vi "Device_connection_info.vi"(11 "Array":string[](array[string])=["COM7", "", "", "COM6"]) -> (3 "Array 3":string[](array[string]))   [LabVIEW 2021]
panel:
  in  "Array 2":string[](array[string])=["Main Crl is not connnected", "Rs485_1 is not connecetd", "RS485_2 is not connected", "RS422 is not connected"]
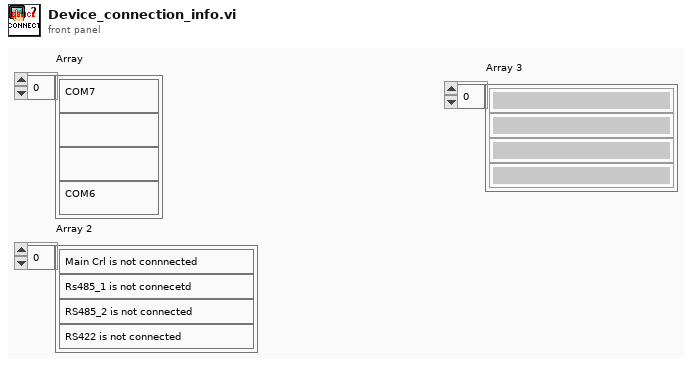
[diagram p1: front panel]
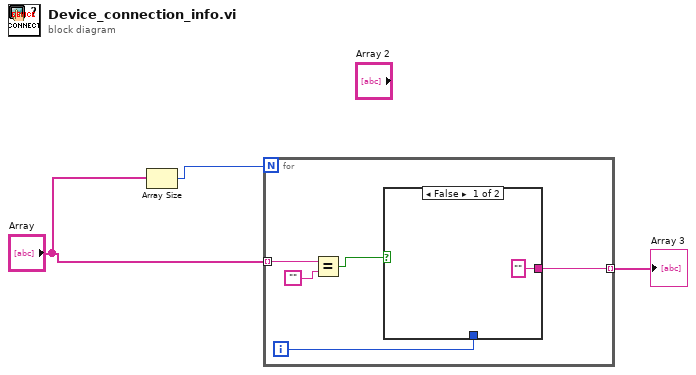
[diagram p0: block diagram]
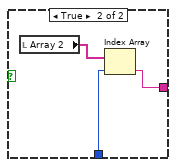
[diagram p2: hidden frame]
diagram:
  n1 = Array Size(array="Array") -> (size(s)=w3:i32)
  n2 = for {
    N: w3 -> [_]
    tunnel: "Array" -> [w8] mode=indexing
    tunnel: [w4] -> w1 mode=indexing
    i -> [w5]
    n3 = Equal?(x=w8, y="") -> (x = y?=w6:bool)
    n4 = case shown="False" w6 {
      tunnel: w5 -> [_ w11]
      tunnel: ["" w10] -> w4
      frame False {
      }
      frame True {
        n5 = local read "Array 2"() -> (w12:string[])
        n6 = Index Array(array=w12, index=w11) -> (element=w10:string)
      }
    }
  }
  "Array 3" <- w1
